vi "Valid Plugin Name.vi"(8 "error in":errorcluster, 10 "requested plugin name":string, 11 "project refnum":refnum<vi>) -> (0 "error out":errorcluster, 3 "valid name?":bool)   [LabVIEW 2021, in "InstrumentStudio Plug-In Editor.lvlib"]
uses:
  InstrumentStudio Plug-In Editor.lvlib
  48953c88-0603-4c13-ba6a-df914321b09e.vi
  <vilib>/Comparison/Equal/Equal Functor/Equal Functor.lvclass
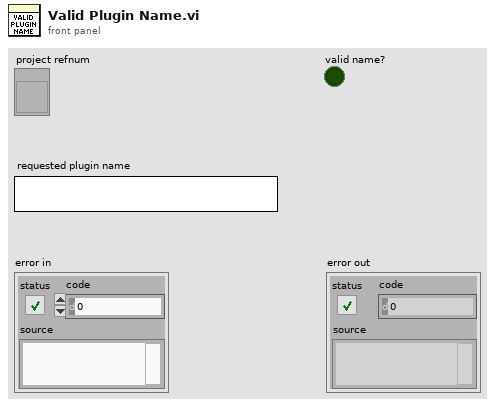
[diagram p1: front panel]
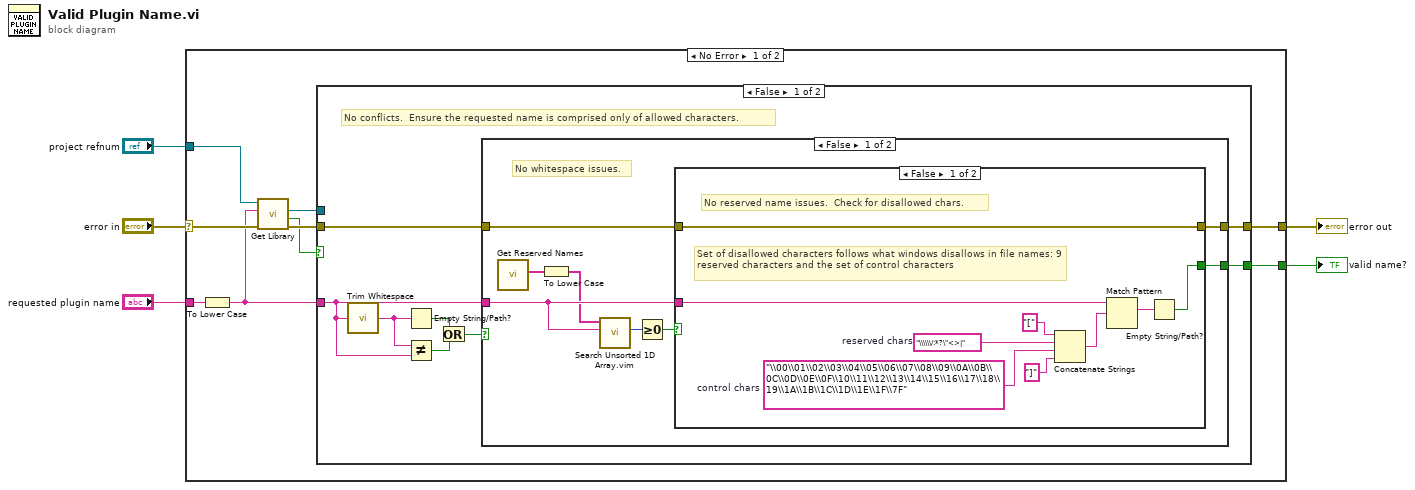
[diagram p0: block diagram]
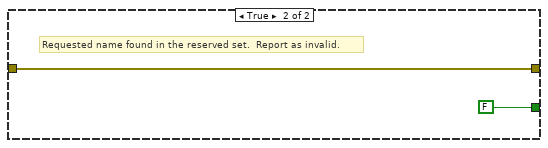
[diagram p2: hidden frame]
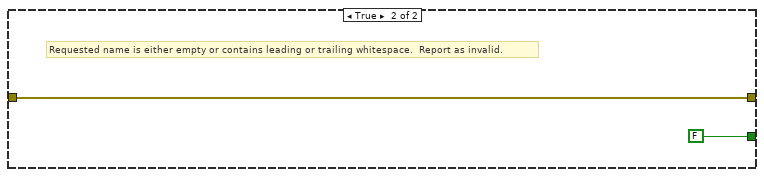
[diagram p3: hidden frame]
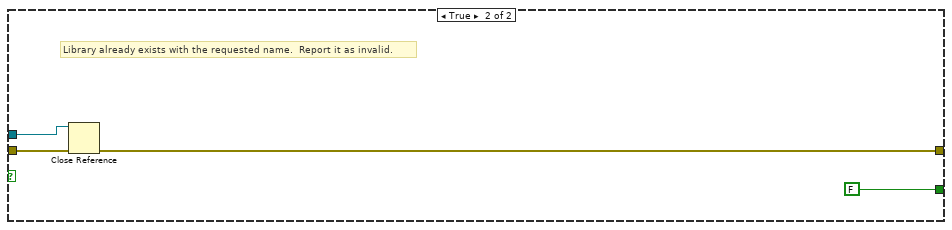
[diagram p4: hidden frame]
diagram:
  n1 = case shown="No Error" "error in" {
    selector: "error in" -> [w14 w48]
    tunnel: [w11 w48] -> w5
    tunnel: [w10 _] -> w4
    tunnel: "project refnum" -> [w9 _]
    tunnel: "requested plugin name" -> [w8 _]
    frame No Error {
      n2 = To Lower Case(string=w8) -> (all lower case string=w7:string)
      n3 = call "Get Library.vi"("error in"=w14, "library name"=w7, "project refnum in"=w9) -> ("error out"=w13:errorcluster, "library found?"=w6:bool, "library refnum"=w12:refnum<vi>)  [unwired: 5 in, 1 out]
      n4 = case shown="False" w6 {
        tunnel: w13 -> [w22 w47]
        tunnel: w12 -> [_ w45]
        tunnel: [w21 w46] -> w11
        tunnel: [w20 FALSE ("Valid Name?")] -> w10
        tunnel: w7 -> [w15 _]
        frame False {
          # "No conflicts.  Ensure the requested name is comprised only of allowed characters."
          n5 = call <vilib>:"Trim Whitespace.vi"("string"=w15) -> ("trimmed string"=w16:string)  [unwired: 1 in]
          n6 = Empty String/Path?(string/path=w16) -> (empty?=w18:bool)
          n7 = Not Equal?(x=w16, y=w15) -> (x != y?=w19:bool)
          n8 = Or(x=w18, y=w19) -> (x .or. y?=w17:bool)
          n9 = case shown="False" w17 {
            tunnel: w15 -> [w24 _]
            tunnel: w22 -> [w30 w43]
            tunnel: [w29 w43] -> w21
            tunnel: [w26 FALSE ("Error if not Found (T)")] -> w20
            frame False {
              # "No whitespace issues."
              n10 = call "Get Reserved Names.vi"() -> ("reserved names"=w25:string[])  [unwired: 11 in]
              n11 = To Lower Case(string=w25) -> (all lower case string=w23:string[])
              n12 = call "Search Unsorted 1D Array.vim"("element"=w24, "unsorted 1D array"=w23) -> ("index of element"=w28:i32)  [unwired: 9 in]
              n13 = Greater Or Equal To 0?(x=w28) -> (x >= 0?=w27:bool)
              n14 = case shown="False" w27 {
                tunnel: w24 -> [w38 _]
                tunnel: w30 -> [w39 w41]
                tunnel: [w39 w41] -> w29
                tunnel: [w32 FALSE ("Error if not Found (T)")] -> w26
                frame False {
                  w31 = "\\00\\01\\02\\03\\04\\05\\06\\07\\08\\09\\0A\\0B\\0C\\0D\\0E\\0F\\10\\11\\12\\13\\14\\15\\16\\17\\18\\19\\1A\\1B\\1C\\1D\\1E\\1F\\7F"  # control chars
                  w37 = "\\\\\\/:*?\"<>|"  # reserved chars
                  # "Set of disallowed characters follows what windows disallows in file names: 9 reserved characters and the set of control characters"
                  # "No reserved name issues.  Check for disallowed chars."
                  n15 = Concatenate Strings("[" ("string"), w37, w31, "]" ("string")) -> (w34:string)
                  n16 = Match Pattern(string=w38, regular expression=w34) -> (match substring=w33:string)  [unwired: 1 in, 3 out]
                  n17 = Empty String/Path?(string/path=w33) -> (empty?=w32:bool)
                }
                frame True {
                  # "Requested name found in the reserved set.  Report as invalid."
                }
              }
            }
            frame True {
              # "Requested name is either empty or contains leading or trailing whitespace.  Report as invalid."
            }
          }
        }
        frame True {
          # "Library already exists with the requested name.  Report it as invalid."
          n18 = Close Reference(reference=w45, error in (no error)=w47) -> (error out=w46:errorcluster)
        }
      }
    }
    frame Error {
    }
  }
  "error out" <- w5
  "valid name?" <- w4
